vi "Style Panel.vi"(0 "VI":path, 1 "Silver":path, 2 "Spec":path, 8 "error in":errorcluster) -> (5 "problems":string[](array[string]), 11 "error out":errorcluster)   [LabVIEW 2020]
doc: "Build tool of the RemoteVI examples (source: tools\\aixml\\Dev\\gen_style_panel.py). Restyles the front panel of a composed VI in place and saves it: the composer only makes generic controls. Run it once on a freshly composed VI (or on one whose controls are all still top-level), with the VI idle. Steps: (1) every row with a Ctl is Replaced by that .ctl under Silver (a path relative to vi.lib\\silver_ctls, e.g. Numeric\\Knob NI_Silver.ctl); wires, data type, enum items and default value stay. (2) Tabs: each tab control gets as many pages as Pages names (Add Page), the page labels, and fixed tabs of Tab Width; with Width above 0 the control - also one that is no tab control, such as a subpanel - is sized through its own pane (Set Scaling Scale Single Object, the window grown by the difference, scaling off again). (3) every row: moved onto page Page of the tab control Tab (Left/Top relative to the tab control) or, with Tab empty and Pane 0 or more, into that pane of the panel (Left/Top in pane coordinates), otherwise placed at Left/Top; Width/Height (0: keep) set the size of a string, button, numeric, the visible area of a multicolumn listbox and the plot area of a graph; Text sets a boolean's text (and centres it); Tip the tip strip; Show Label and Visible. (4) Window sets the panel bounds and the origin to 0,0. Controls are found anywhere on the panel by label (Find Controls). problems lists every row whose steps returned an error, with the code; the run goes on."
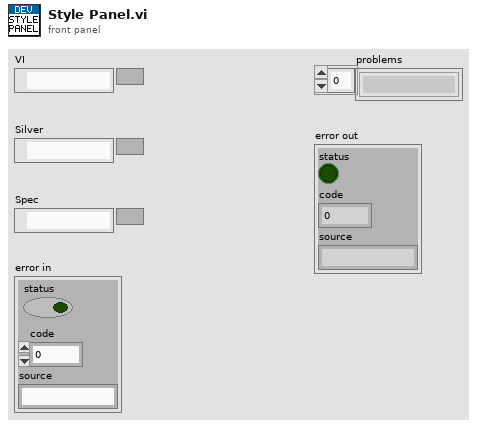
[diagram p1: front panel]
types:
  T1 = cluster{"Rows":cluster{"Label":string, "Ctl":string, "Tab":string, "Page":i32, "Pane":i32, "Left":i32, "Top":i32, "Width":i32, "Height":i32, "Text":string, "Tip":string, "Show Label":bool, "Visible":bool}[], "Tabs":cluster{"Tab":string, "Pages":string[], "Tab Width":i32, "Width":i32, "Height":i32}[], "Window":cluster{"Left":i32, "Top":i32, "Right":i32, "Bottom":i32}, "Splitters":i32[]}
  T2 = cluster{"Label":string, "Ctl":string, "Tab":string, "Page":i32, "Pane":i32, "Left":i32, "Top":i32, "Width":i32, "Height":i32, "Text":string, "Tip":string, "Show Label":bool, "Visible":bool}[]
  T3 = cluster{"Tab":string, "Pages":string[], "Tab Width":i32, "Width":i32, "Height":i32}[]
  T4 = cluster{"Left":i32, "Top":i32, "Right":i32, "Bottom":i32}
  T5 = enum16{"No Scaling", "Scale All Objects", "Scale Single Object"}
  T6 = typedef "LVBoundsTypeDef.ctl" = cluster{"Width":u32, "Height":u32}
  T7 = typedef "LVRectTypeDef.ctl" = cluster{"Left":i16, "Top":i16, "Right":i16, "Bottom":i16}
  T8 = typedef "LVPositionTypeDef.ctl" = cluster{"Left":i32, "Top":i32}
  T9 = typedef "LVPointTypeDef.ctl" = cluster{"Horizontal":i16, "Vertical":i16}
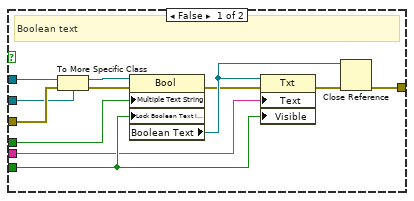
[diagram p3: hidden frame]
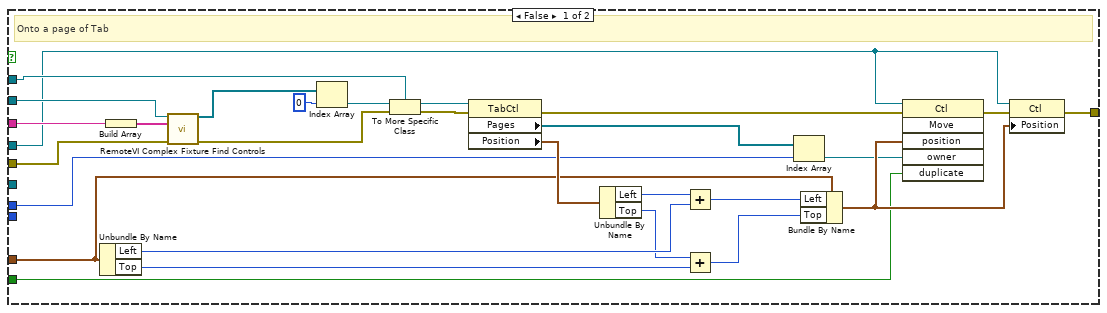
[diagram p5: hidden frame]
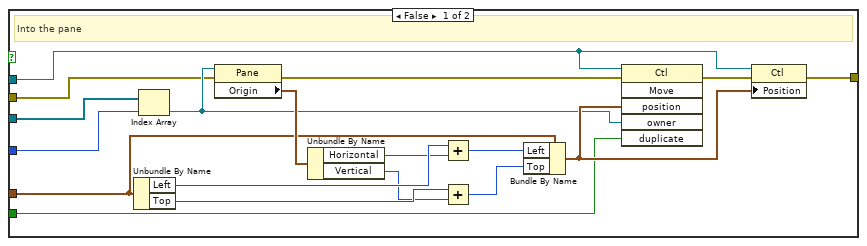
[diagram p6: hidden frame]
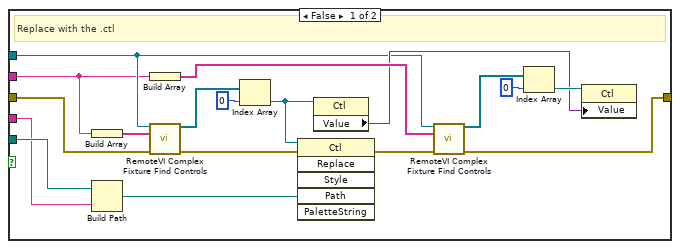
[diagram p8: hidden frame]
diagram:
  w32 = refnum<vi> refnum  # boolean class
  w31 = refnum<vi> refnum  # graph class
  w30 = refnum<vi> refnum  # string class
  w27 = 2  # fixed tabs
  w26 = refnum<vi> refnum  # tab class
  w23 = FALSE  # false
  w22 = TRUE  # true
  w21 = FALSE  # no duplicate
  w7 = T1 {"Rows"=[], "Tabs"=[], "Window"={"Left"=0, "Top"=0, "Right"=0, "Bottom"=0}, "Splitters"=[]}  # spec type
  # "Replace, tabs, place, window, save"
  n1 = Read from Text File(file (use dialog)="Spec", error in="error in") -> (text=w4:string, error out=w5:errorcluster)  [unwired: 2 in, 2 out]
  n2 = Unflatten From XML(xml string=w4, type=w7, error in (no error)=w5) -> (value=w8:T1, error out=w9:errorcluster)
  n3 = Open VI Reference(vi path="VI", error in (no error)=w9) -> (vi reference=w14:refnum<vi>, error out=w15:errorcluster)  [unwired: 4 in]
  n4 = property class="VI"(reference=w14, error in=w15) -> (error out=w16:errorcluster, "Front Panel"=w17:refnum<vi>)  [unwired: 1 out]
  n5 = Unbundle By Name(w8) -> ("Rows"=w10:T2, "Tabs"=w11:T3, "Window"=w12:T4, "Splitters"=w13:i32[])
  n6 = property class="Pnl"(reference=w17, error in=w16) -> (error out=w18:errorcluster, "Panes[]"=w19:refnum<vi>[])  [unwired: 1 out]
  n7 = property class="Pnl"(reference=w17, error in=w18) -> ("Splitters[]"=w20:refnum<vi>[])  [unwired: 2 out]
  n8 = Unbundle By Name(w12) -> ("Right"=w36:i32)
  n9 = Greater Than 0?(x=w36) -> (x > 0?=w37:bool)
  n10 = for {
    tunnel: w13 -> [w43] mode=indexing
    tunnel: w20 -> [w42] mode=indexing
    # "Each splitter bar to its position"
    n11 = property class="Splitter"(reference=w42, "Position"=w43) -> ()  [unwired: 1 in, 2 out]
  }
  n12 = for {
    tunnel: "Silver" -> [w46]
    tunnel: w10 -> [w44] mode=indexing
    tunnel: w17 -> [w45]
    shift-right: [w48] -> w24
    shift-left: w18 -> [w47]
    tunnel: [w56] -> w25 mode=indexing
    # "Replace each control that has a Ctl"
    n13 = Unbundle By Name(w44) -> ("Label"=w49:string, "Ctl"=w50:string)
    n14 = Empty String/Path?(string/path=w50) -> (empty?=w51:bool)
    n15 = case shown="True" w51 {
      tunnel: w46 -> [w60 _]
      tunnel: w49 -> [w57 _]
      tunnel: w50 -> [w58 _]
      tunnel: w45 -> [w59 _]
      tunnel: w47 -> [w61 w75]
      tunnel: [w72 w75] -> w52
      frame False {
        # "Replace with the .ctl"
        n16 = Build Array(w57) -> (w62:string[])
        n17 = Build Path(base path=w60, name or relative path=w58) -> (appended path=w67:path)
        n18 = Build Array(w57) -> (w70:string[])
        n19 = call "RemoteVI Complex Fixture Find Controls.vi"("Panel"=w59, "labels"=w62, "error in"=w61) -> ("Controls"=w63:refnum<vi>[], "error out"=w64:errorcluster)  [unwired: 11 in]
        n20 = Index Array(array=w63, index=0) -> (element=w66:refnum<vi>)
        n21 = invoke class="Ctl" method="Replace"(reference=w66, error in=w64, "Path"=w67) -> (error out=w69:errorcluster)  [unwired: 3 in, 5 out]
        n22 = property class="Ctl"(reference=w66) -> ("Value"=w68:variant)  [unwired: 1 in, 2 out]
        n23 = call "RemoteVI Complex Fixture Find Controls.vi"("Panel"=w59, "labels"=w70, "error in"=w69) -> ("Controls"=w71:refnum<vi>[], "error out"=w72:errorcluster)  [unwired: 11 in]
        n24 = Index Array(array=w71, index=0) -> (element=w74:refnum<vi>)
        n25 = property class="Ctl"(reference=w74, "Value"=w68) -> ()  [unwired: 1 in, 2 out]
      }
      frame True {
        # "No Ctl: keep"
      }
    }
    n26 = Unbundle By Name(w52) -> ("code"=w53:i32, "source"=w54:string)
    n27 = call <vilib>:"Clear Errors.vi"("error in (no error)"=w52) -> ("error out"=w48:errorcluster)  [unwired: 5 in, 1 out]
    n28 = Format Into String(format string="%s Replace %d %s", w49, w53, w54) -> (resulting string=w56:string)  [unwired: 2 in, 1 out]
  }
  n29 = for {
    tunnel: w26 -> [w78]
    tunnel: w27 -> [w79]
    tunnel: w11 -> [w76] mode=indexing
    tunnel: w14 -> [w80]
    tunnel: w17 -> [w77]
    tunnel: w19 -> [w81]
    shift-right: [w83] -> w28
    shift-left: w24 -> [w82]
    tunnel: [w115] -> w29 mode=indexing
    # "Pages of each tab control"
    n30 = Unbundle By Name(w76) -> ("Tab"=w84:string, "Pages"=w85:string[], "Tab Width"=w86:i32, "Width"=w87:i32, "Height"=w88:i32)
    n31 = Array Size(array=w85) -> (size(s)=w101:i32)
    n32 = Build Array(w84) -> (w89:string[])
    n33 = call "RemoteVI Complex Fixture Find Controls.vi"("Panel"=w77, "labels"=w89, "error in"=w82) -> ("Controls"=w90:refnum<vi>[], "error out"=w91:errorcluster)  [unwired: 11 in]
    n34 = Index Array(array=w90, index=0) -> (element=w93:refnum<vi>)
    n35 = To More Specific Class(target class=w78, reference=w93, error in=w91) -> (specific class reference=w94:refnum<vi>, error out=w95:errorcluster)
    n36 = Bundle By Name(cluster=cluster{"Width":i32, "Height":i32} {"Width"=110, "Height"=24}, "Width"=w86, "Height"=24) -> (w98:cluster{"Width":i32, "Height":i32})
    n37 = property class="TabCtl"(reference=w94, error in=w95, "Tab Size"=w79, "Fixed Tab Dimension"=w98) -> (error out=w99:errorcluster, "Pages"=w100:refnum<vi>[])  [unwired: 1 out]
    n38 = Array Size(array=w100) -> (size(s)=w102:i32)
    n39 = Subtract(x=w101, y=w102) -> (x-y=w103:i32)
    n40 = Greater Than 0?(x=w87) -> (x > 0?=w108:bool)
    n41 = for {
      N: w103 -> [_]
      tunnel: w94 -> [w153]
      shift-right: [w155] -> w104
      shift-left: w99 -> [w154]
      # "Add the missing pages"
      n42 = invoke class="TabCtl" method="Add Page"(reference=w153, error in=w154, "Page"=0, "After"=TRUE) -> (error out=w155:errorcluster)  [unwired: 1 in, 4 out]
    }
    n43 = property class="TabCtl"(reference=w94, error in=w104) -> (error out=w105:errorcluster, "Pages"=w106:refnum<vi>[])  [unwired: 1 out]
    n44 = for {
      tunnel: w85 -> [w150] mode=indexing
      tunnel: w106 -> [w149] mode=indexing
      shift-right: [w152] -> w107
      shift-left: w105 -> [w151]
      # "Name each page"
      n45 = property class="Page"(reference=w149, "TabCaption"=w150) -> ()  [unwired: 1 in, 2 out]
      n46 = property class="Page"(reference=w149, error in=w151, "Page Label"=w150) -> (error out=w152:errorcluster)  [unwired: 1 out]
    }
    n47 = call <vilib>:"Clear Errors.vi"("error in (no error)"=w107) -> ("error out"=w109:errorcluster)  [unwired: 5 in, 1 out]
    n48 = case shown="True" w108 {
      tunnel: w80 -> [_ w118]
      tunnel: w87 -> [_ w119]
      tunnel: w88 -> [_ w120]
      tunnel: w81 -> [_ _]
      tunnel: w93 -> [_ w117]
      tunnel: w109 -> [w116 w121]
      tunnel: [w116 w148] -> w110
      frame False {
        # "Keep the size"
      }
      frame True {
        w142 = 40
        # "Scale the tab control with the pane once"
        n49 = property class="Ctl"(reference=w117, error in=w121) -> (error out=w123:errorcluster, "OwningPane"=w122:refnum<vi>)  [unwired: 1 out]
        n50 = invoke class="Pane" method="Set Scaling"(reference=w122, error in=w123, "ScalingMode"=T5."Scale Single Object", "ScalableObj"=w117) -> (error out=w126:errorcluster)  [unwired: 1 in, 4 out]
        n51 = property class="Ctl"(reference=w117, error in=w126) -> (error out=w127:errorcluster, "Bounds"=w128:T6)  [unwired: 1 out]
        n52 = property class="VI"(reference=w118, error in=w127) -> (error out=w131:errorcluster, "Front Panel Window:Panel Bounds"=w132:T7)  [unwired: 1 out]
        n53 = Unbundle By Name(w128) -> ("Width"=w129:u32, "Height"=w130:u32)
        n54 = Unbundle By Name(w132) -> ("Left"=w133:i16, "Top"=w134:i16, "Right"=w135:i16, "Bottom"=w136:i16)
        n55 = Subtract(x=w119, y=w129) -> (x-y=w137:u32)
        n56 = Subtract(x=w120, y=w130) -> (x-y=w138:u32)
        n57 = Subtract(x=w135, y=w133) -> (x-y=w139:i16)
        n58 = Subtract(x=w136, y=w134) -> (x-y=w140:i16)
        n59 = Add(x=w139, y=w137) -> (x+y=w141:u32)
        n60 = Add(x=w140, y=w138) -> (x+y=w144:u32)
        n61 = Add(x=w144, y=w142) -> (x+y=w145:u32)
        n62 = Bundle By Name(cluster=w132, "Left"=0, "Top"=w142, "Right"=w141, "Bottom"=w145) -> (w146:T7)
        n63 = property class="VI"(reference=w118, error in=w131, "Front Panel Window:Panel Bounds"=w146) -> (error out=w147:errorcluster)  [unwired: 1 out]
        n64 = invoke class="Pane" method="Set Scaling"(reference=w122, error in=w147, "ScalingMode"=T5."No Scaling", "ScalableObj"=w117) -> (error out=w148:errorcluster)  [unwired: 1 in, 4 out]
      }
    }
    n65 = Merge Errors(w110, w107) -> (w111:errorcluster)
    n66 = Unbundle By Name(w111) -> ("code"=w112:i32, "source"=w113:string)
    n67 = call <vilib>:"Clear Errors.vi"("error in (no error)"=w111) -> ("error out"=w83:errorcluster)  [unwired: 5 in, 1 out]
    n68 = Format Into String(format string="%s Tabs %d %s", w84, w112, w113) -> (resulting string=w115:string)  [unwired: 2 in, 1 out]
  }
  n69 = case shown="True" w37 {
    tunnel: w14 -> [_ w159]
    tunnel: w12 -> [_ w160]
    tunnel: w28 -> [w158 w161]
    tunnel: [w158 w164] -> w33
    frame False {
      # "Keep the window"
    }
    frame True {
      w163 = FALSE
      # "Window bounds, origin 0,0"
      n70 = property class="VI"(reference=w159, error in=w161, "Front Panel Window:Show Menu Bar"=w163, "Tool Bar:Visible"=w163, "Front Panel Window:Show Scroll Bars"=w163, "Front Panel Window:Panel Bounds"=w160, "Front Panel Window:Origin"=cluster{"Horizontal":i32, "Vertical":i32} {"Horizontal"=0, "Vertical"=0}) -> (error out=w164:errorcluster)  [unwired: 1 out]
    }
  }
  n71 = for {
    tunnel: w26 -> [w168]
    tunnel: w21 -> [w169]
    tunnel: w30 -> [w170]
    tunnel: w31 -> [w171]
    tunnel: w32 -> [w172]
    tunnel: w22 -> [w173]
    tunnel: w23 -> [w174]
    tunnel: w10 -> [w165] mode=indexing
    tunnel: w17 -> [w166]
    tunnel: w19 -> [w167]
    shift-right: [w176] -> w34
    shift-left: w33 -> [w175]
    tunnel: [w208] -> w35 mode=indexing
    # "Move and set each control"
    n72 = Unbundle By Name(w165) -> ("Label"=w177:string, "Tab"=w178:string, "Page"=w179:i32, "Pane"=w180:i32, "Left"=w181:i32, "Top"=w182:i32, "Width"=w183:i32, "Height"=w184:i32, "Text"=w185:string, "Tip"=w186:string, "Show Label"=w187:bool, "Visible"=w188:bool)
    n73 = Empty String/Path?(string/path=w185) -> (empty?=w202:bool)
    n74 = Empty String/Path?(string/path=w178) -> (empty?=w196:bool)
    n75 = Build Array(w177) -> (w189:string[])
    n76 = call "RemoteVI Complex Fixture Find Controls.vi"("Panel"=w166, "labels"=w189, "error in"=w175) -> ("Controls"=w190:refnum<vi>[], "error out"=w191:errorcluster)  [unwired: 11 in]
    n77 = Bundle By Name(cluster=cluster{"Left":i32, "Top":i32} {"Left"=0, "Top"=0}, "Left"=w181, "Top"=w182) -> (w195:cluster{"Left":i32, "Top":i32})
    n78 = Index Array(array=w190, index=0) -> (element=w193:refnum<vi>)
    n79 = Greater Than 0?(x=w183) -> (x > 0?=w198:bool)
    n80 = case shown="True" w196 {
      tunnel: w168 -> [w278 _]
      tunnel: w169 -> [w279 w305]
      tunnel: w178 -> [w275 _]
      tunnel: w179 -> [w276 _]
      tunnel: w180 -> [_ w303]
      tunnel: w166 -> [w277 _]
      tunnel: w195 -> [w274 w302]
      tunnel: w167 -> [_ w304]
      tunnel: w191 -> [w273 w301]
      tunnel: w193 -> [w272 w300]
      tunnel: [w299 w307] -> w197
      frame False {
        # "Onto a page of Tab"
        n81 = Unbundle By Name(w274) -> ("Left"=w293:i32, "Top"=w294:i32)
        n82 = Build Array(w275) -> (w280:string[])
        n83 = call "RemoteVI Complex Fixture Find Controls.vi"("Panel"=w277, "labels"=w280, "error in"=w273) -> ("Controls"=w281:refnum<vi>[], "error out"=w282:errorcluster)  [unwired: 11 in]
        n84 = Index Array(array=w281, index=0) -> (element=w284:refnum<vi>)
        n85 = To More Specific Class(target class=w278, reference=w284, error in=w282) -> (specific class reference=w285:refnum<vi>, error out=w286:errorcluster)
        n86 = property class="TabCtl"(reference=w285, error in=w286) -> (error out=w287:errorcluster, "Pages"=w288:refnum<vi>[], "Position"=w289:T8)  [unwired: 1 out]
        n87 = Unbundle By Name(w289) -> ("Left"=w291:i32, "Top"=w292:i32)
        n88 = Add(x=w291, y=w293) -> (x+y=w295:i32)
        n89 = Add(x=w292, y=w294) -> (x+y=w296:i32)
        n90 = Index Array(array=w288, index=w276) -> (element=w290:refnum<vi>)
        n91 = Bundle By Name(cluster=w274, "Left"=w295, "Top"=w296) -> (w297:cluster{"Left":i32, "Top":i32})
        n92 = invoke class="Ctl" method="Move"(reference=w272, error in=w287, "position"=w297, "owner"=w290, "duplicate"=w279) -> (error out=w298:errorcluster)  [unwired: 1 in, 5 out]
        n93 = property class="Ctl"(reference=w272, error in=w298, "Position"=w297) -> (error out=w299:errorcluster)  [unwired: 1 out]
      }
      frame True {
        # "Tab empty: pane or panel"
        n94 = Less Than 0?(x=w303) -> (x < 0?=w306:bool)
        n95 = case shown="True" w306 {
          tunnel: w305 -> [w313 _]
          tunnel: w303 -> [w311 _]
          tunnel: w302 -> [w310 w328]
          tunnel: w304 -> [w312 _]
          tunnel: w301 -> [w309 w327]
          tunnel: w300 -> [w308 w326]
          tunnel: [w325 w329] -> w307
          frame False {
            # "Into the pane"
            n96 = Unbundle By Name(w310) -> ("Left"=w319:i32, "Top"=w320:i32)
            n97 = Index Array(array=w312, index=w311) -> (element=w314:refnum<vi>)
            n98 = property class="Pane"(reference=w314, error in=w309) -> (error out=w315:errorcluster, "Origin"=w316:T9)  [unwired: 1 out]
            n99 = Unbundle By Name(w316) -> ("Horizontal"=w317:i16, "Vertical"=w318:i16)
            n100 = Add(x=w319, y=w317) -> (x+y=w321:i32)
            n101 = Add(x=w320, y=w318) -> (x+y=w322:i32)
            n102 = Bundle By Name(cluster=w310, "Left"=w321, "Top"=w322) -> (w323:cluster{"Left":i32, "Top":i32})
            n103 = invoke class="Ctl" method="Move"(reference=w308, error in=w315, "position"=w323, "owner"=w314, "duplicate"=w313) -> (error out=w324:errorcluster)  [unwired: 1 in, 5 out]
            n104 = property class="Ctl"(reference=w308, error in=w324, "Position"=w323) -> (error out=w325:errorcluster)  [unwired: 1 out]
          }
          frame True {
            # "No pane: place"
            n105 = property class="Ctl"(reference=w326, error in=w327, "Position"=w328) -> (error out=w329:errorcluster)  [unwired: 1 out]
          }
        }
      }
    }
    n106 = Bundle By Name(cluster=cluster{"Width":i32, "Height":i32} {"Width"=0, "Height"=0}, "Width"=w183, "Height"=w184) -> (w200:cluster{"Width":i32, "Height":i32})
    n107 = case shown="True" w198 {
      tunnel: w170 -> [_ _]
      tunnel: w171 -> [_ _]
      tunnel: w200 -> [_ w224]
      tunnel: w193 -> [_ w223]
      tunnel: w197 -> [w222 w225]
      tunnel: [w222 w225] -> w201
      frame False {
        # "No size"
      }
      frame True {
        w270 = u8 1
        w265 = u32 3884370
        w261 = refnum<vi> refnum  # WaveformGraph
        w254 = refnum<vi> refnum  # Table
        w251 = refnum<vi> refnum  # MulticolumnListbox
        w248 = refnum<vi> refnum  # WaveformGraph
        w245 = refnum<vi> refnum  # NamedNumeric
        w242 = refnum<vi> refnum  # Digital
        w239 = refnum<vi> refnum  # NumericWithScale
        w236 = refnum<vi> refnum  # Path
        w233 = refnum<vi> refnum  # String
        w230 = refnum<vi> refnum  # Boolean
        # "Size by class"
        n108 = Unbundle By Name(w224) -> ("Width"=w226:i32, "Height"=w227:i32)
        n109 = To More Specific Class(target class=w254, reference=w223) -> (specific class reference=w255:refnum<vi>, error out=w256:errorcluster)  [unwired: 1 in]
        n110 = To More Specific Class(target class=w242, reference=w223) -> (specific class reference=w243:refnum<vi>, error out=w244:errorcluster)  [unwired: 1 in]
        n111 = Quotient & Remainder(x=w227, y=20) -> (floor(x/y)=w259:i32)  [unwired: 1 out]
        n112 = Quotient & Remainder(x=w226, y=120) -> (floor(x/y)=w260:i32)  [unwired: 1 out]
        n113 = Bundle By Name(cluster=cluster{"Width":u32, "Height":u32} {"Width"=0, "Height"=0}, "Width"=w226, "Height"=w227) -> (w229:cluster{"Width":u32, "Height":u32})
        n114 = property class="Tbl"(reference=w255, error in=w256, "Number of Rows"=w259, "Number of Columns"=w260) -> ()  [unwired: 2 out]
        n115 = property class="DigNum"(reference=w243, error in=w244, "Text Width"=w226) -> ()  [unwired: 2 out]
        n116 = To More Specific Class(target class=w261, reference=w223) -> (specific class reference=w262:refnum<vi>, error out=w263:errorcluster)  [unwired: 1 in]
        n117 = To More Specific Class(target class=w230, reference=w223) -> (specific class reference=w231:refnum<vi>, error out=w232:errorcluster)  [unwired: 1 in]
        n118 = To More Specific Class(target class=w233, reference=w223) -> (specific class reference=w234:refnum<vi>, error out=w235:errorcluster)  [unwired: 1 in]
        n119 = To More Specific Class(target class=w236, reference=w223) -> (specific class reference=w237:refnum<vi>, error out=w238:errorcluster)  [unwired: 1 in]
        n120 = To More Specific Class(target class=w239, reference=w223) -> (specific class reference=w240:refnum<vi>, error out=w241:errorcluster)  [unwired: 1 in]
        n121 = To More Specific Class(target class=w248, reference=w223) -> (specific class reference=w249:refnum<vi>, error out=w250:errorcluster)  [unwired: 1 in]
        n122 = To More Specific Class(target class=w245, reference=w223) -> (specific class reference=w246:refnum<vi>, error out=w247:errorcluster)  [unwired: 1 in]
        n123 = property class="Bool"(reference=w231, error in=w232, "Button Size"=w229) -> ()  [unwired: 2 out]
        n124 = property class="Str"(reference=w234, error in=w235, "Size"=w229) -> ()  [unwired: 2 out]
        n125 = property class="Path"(reference=w237, error in=w238, "Size"=w229) -> ()  [unwired: 2 out]
        n126 = property class="NumWthScl"(reference=w240, error in=w241, "Housing Size"=w229) -> ()  [unwired: 2 out]
        n127 = property class="WFGraph"(reference=w249, error in=w250, "Plot Area:Size"=w224) -> ()  [unwired: 2 out]
        n128 = property class="NmdNum"(reference=w246, error in=w247, "Named Numeric Size"=w229) -> ()  [unwired: 2 out]
        n129 = To More Specific Class(target class=w251, reference=w223) -> (specific class reference=w252:refnum<vi>, error out=w253:errorcluster)  [unwired: 1 in]
        n130 = property class="MCListbox"(reference=w252, error in=w253, "Bounds:Area Width"=w226, "Bounds:Area Height"=w227) -> ()  [unwired: 2 out]
        n131 = property class="WFGraph"(reference=w262, error in=w263, "Plot Area:Colors:BG Color"=u32 2304563, "Grid Colors:X Color"=w265, "Grid Colors:Y Color"=w265, "Legend Visible"=FALSE) -> (error out=w267:errorcluster, "X Scale"=w268:refnum<vi>, "Y Scale"=w269:refnum<vi>)  [unwired: 1 out]
        n132 = property class="GrphScl"(reference=w268, error in=w267, "Scale Fit"=w270) -> (error out=w271:errorcluster)  [unwired: 1 out]
        n133 = property class="GrphScl"(reference=w269, error in=w271, "Scale Fit"=w270) -> ()  [unwired: 2 out]
      }
    }
    n134 = case shown="True" w202 {
      tunnel: w172 -> [w211 _]
      tunnel: w173 -> [w212 _]
      tunnel: w174 -> [w213 _]
      tunnel: w185 -> [w210 _]
      tunnel: w193 -> [w209 _]
      tunnel: w201 -> [w214 w221]
      tunnel: [w220 w221] -> w203
      frame False {
        # "Boolean text"
        n135 = To More Specific Class(target class=w211, reference=w209, error in=w214) -> (specific class reference=w215:refnum<vi>, error out=w216:errorcluster)
        n136 = property class="Bool"(reference=w215, error in=w216, "Multiple Text String"=w213, "Lock Boolean Text In Center"=w212) -> (error out=w217:errorcluster, "Boolean Text"=w218:refnum<vi>)  [unwired: 1 out]
        n137 = property class="Txt"(reference=w218, error in=w217, "Text"=w210, "Visible"=w212) -> (error out=w219:errorcluster)  [unwired: 1 out]
        n138 = Close Reference(reference=w218, error in (no error)=w219) -> (error out=w220:errorcluster)
      }
      frame True {
        # "No text"
      }
    }
    n139 = property class="Ctl"(reference=w193, error in=w203, "TipStrip"=w186, "Label.Visible"=w187, "Visible"=w188) -> (error out=w204:errorcluster)  [unwired: 1 out]
    n140 = Unbundle By Name(w204) -> ("code"=w205:i32, "source"=w206:string)
    n141 = call <vilib>:"Clear Errors.vi"("error in (no error)"=w204) -> ("error out"=w176:errorcluster)  [unwired: 5 in, 1 out]
    n142 = Format Into String(format string="%s Place %d %s", w177, w205, w206) -> (resulting string=w208:string)  [unwired: 2 in, 1 out]
  }
  n143 = invoke class="VI" method="Default Vals.Make Curr Default"(reference=w14, error in=w34) -> (error out=w38:errorcluster)  [unwired: 1 in, 2 out]
  n144 = Build Array (concatenate)(w25, w29, w35) -> (→"problems":string[])
  n145 = invoke class="VI" method="Save.Instrument"(reference=w14, error in=w38) -> (error out=w39:errorcluster)  [unwired: 4 in, 5 out]
  n146 = Close Reference(reference=w14, error in (no error)=w39) -> (error out=→"error out":errorcluster)
